vi "Control Path.vi"(11 "ButtonControlEditorPanel in":refnum<class "NumericButtonEditorPanel.lvclass">) -> (2 "Control Path":path[](array[path]))   [LabVIEW 2025, in "VolatusGUIControls.lvlib" / "NumericButtonEditorPanel.lvclass"]
uses:
  NumericButtonEditorPanel.lvclass
  NumericButtonEditorPanel.lvclass/NumericButtonEditorPanel.ctl
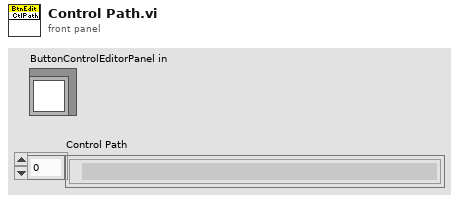
[diagram p1: front panel]
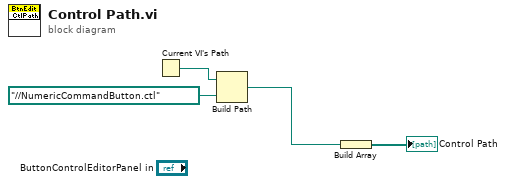
[diagram p0: block diagram]
diagram:
  n1 = Current VI's Path() -> (path=w4:path)
  n2 = Build Path(base path=w4, name or relative path=path "../../NumericCommandButton.ctl") -> (appended path=w2:path)
  n3 = Build Array(w2) -> (→"Control Path":path[])
